vi "Hide SubVI Labels.vi"(8 "error in":errorcluster, 10 "Project Root Folder":path, 11 "IProject Manager in":refnum<class "IProject Manager.lvclass">) -> (0 "error out":errorcluster, 3 "IProject Manager out":refnum<class "IProject Manager.lvclass">)   [LabVIEW 2026, in "IProject Manager.lvclass"]
doc: "This VI iterates through all VIs in the project and hides Labels of Subvis in the block diagram."
uses:
  IProject Manager.lvclass
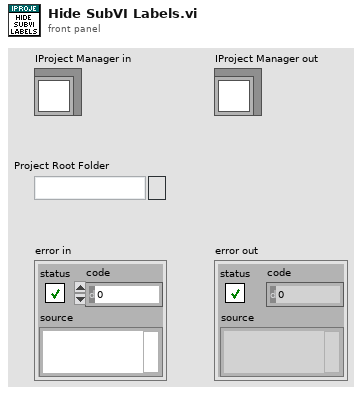
[diagram p1: front panel]
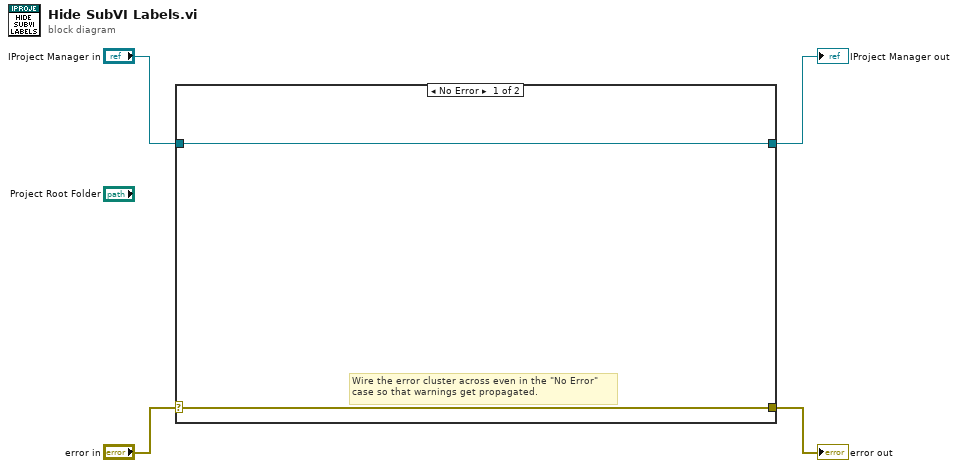
[diagram p0: block diagram]
diagram:
  n1 = case shown="No Error" "error in" {
    selector: "error in" -> [w6 w8]
    tunnel: [w6 w8] -> w3
    tunnel: [w5 w7] -> w1
    tunnel: "IProject Manager in" -> [w5 w7]
    frame No Error {
      # "Wire the error cluster across even in the \"No Error\"\ncase so that warnings get propagated."
    }
    frame Error {
    }
  }
  "error out" <- w3
  "IProject Manager out" <- w1
